vi "ArmPathLength.vi"(4 "ArmPathIn":T1[](array[typedef])) -> (0 "Path Length":dbl, 1 "ArmPathOut":T1[](array[typedef]), 2 "IndexedPathLength":dbl[](array[numeric]))   [LabVIEW 2017]
uses:
  TypeDefs/ArmCoordinate.ctl
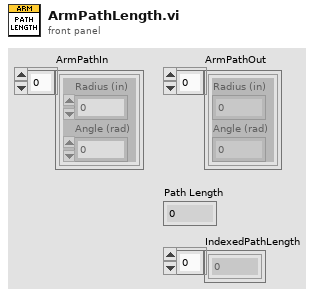
[diagram p1: front panel]
types:
  T1 = typedef "ArmCoordinate.ctl" = cluster{"Radius (in)":dbl, "Angle (rad)":dbl}
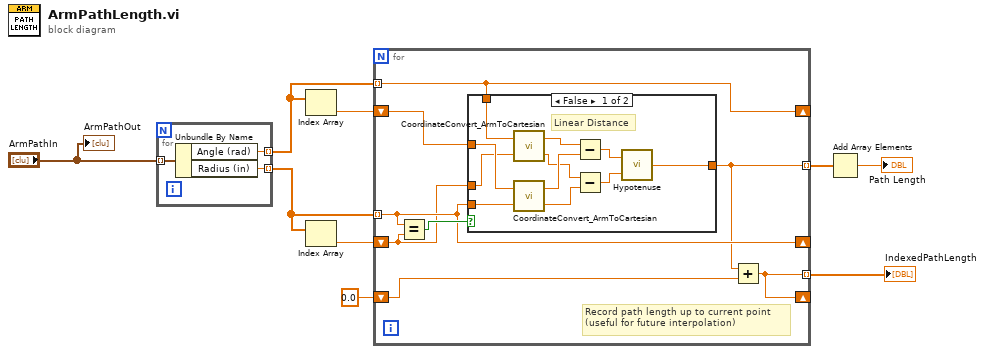
[diagram p0: block diagram]
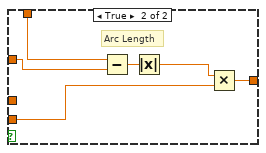
[diagram p2: hidden frame]
diagram:
  n1 = for {
    tunnel: "ArmPathIn" -> [w12] mode=indexing
    tunnel: [w11] -> w3 mode=indexing
    tunnel: [w10] -> w2 mode=indexing
    n2 = Unbundle By Name(w12) -> ("Angle (rad)"=w11:dbl, "Radius (in)"=w10:dbl)
  }
  n3 = Index Array(array=w3) -> (element=w8:dbl)  [unwired: 1 in]
  n4 = Index Array(array=w2) -> (element=w7:dbl)  [unwired: 1 in]
  n5 = for {
    tunnel: w3 -> [w19] mode=indexing
    tunnel: w2 -> [w17] mode=indexing
    shift-right: [w17] -> _
    shift-left: w7 -> [w16]
    shift-right: [w19] -> _
    shift-left: w8 -> [w18]
    tunnel: [w14] -> w6 mode=indexing
    shift-right: [w15] -> _
    shift-left: 0.0 -> [w13]
    tunnel: [w15] -> w4 mode=indexing
    # "Record path length up to current point\n(useful for future interpolation)"
    n6 = Equal?(x=w17, y=w16) -> (x = y?=w20:bool)
    n7 = case shown="False" w20 {
      tunnel: w19 -> [w24 w35]
      tunnel: w16 -> [w22 _]
      tunnel: w17 -> [w21 w32]
      tunnel: [w25 w36] -> w14
      tunnel: w18 -> [w23 w34]
      frame False {
        # "Linear Distance"
        n8 = call "CoordinateConvert_ArmToCartesian.vi"("Radius (in)"=w22, "Angle (rad)"=w24) -> ("Y (in)"=w29:dbl, "X (in)"=w31:dbl)
        n9 = call "CoordinateConvert_ArmToCartesian.vi"("Radius (in)"=w21, "Angle (rad)"=w23) -> ("Y (in)"=w28:dbl, "X (in)"=w30:dbl)
        n10 = Subtract(x=w31, y=w30) -> (x-y=w27:dbl)
        n11 = Subtract(x=w29, y=w28) -> (x-y=w26:dbl)
        n12 = call "Hypotenuse.vi"("Y"=w26, "X"=w27) -> ("Hypotenuse"=w25:dbl)
      }
      frame True {
        # "Arc Length"
        n13 = Subtract(x=w35, y=w34) -> (x-y=w37:dbl)
        n14 = Absolute Value(x=w37) -> (abs(x)=w33:dbl)
        n15 = Multiply(x=w33, y=w32) -> (x*y=w36:dbl)
      }
    }
    n16 = Add(x=w14, y=w13) -> (x+y=w15:dbl)
  }
  "IndexedPathLength" <- w4
  n17 = Add Array Elements(numeric array=w6) -> (sum=→"Path Length":dbl)
  "ArmPathOut" <- "ArmPathIn"
